vi "Variable glob alertes min-max temperatures.vi"() -> ()   [LabVIEW 2022 SP3]
panel:
  out "Groupe ON":bool[](array[boolean])
  out "Liste min/max temp":string[](array[string])
  in  "groupes min max temp":T1(array[cluster])
  in  "Al temp min/max en cours":bool
  # "Alertes min/max températures"
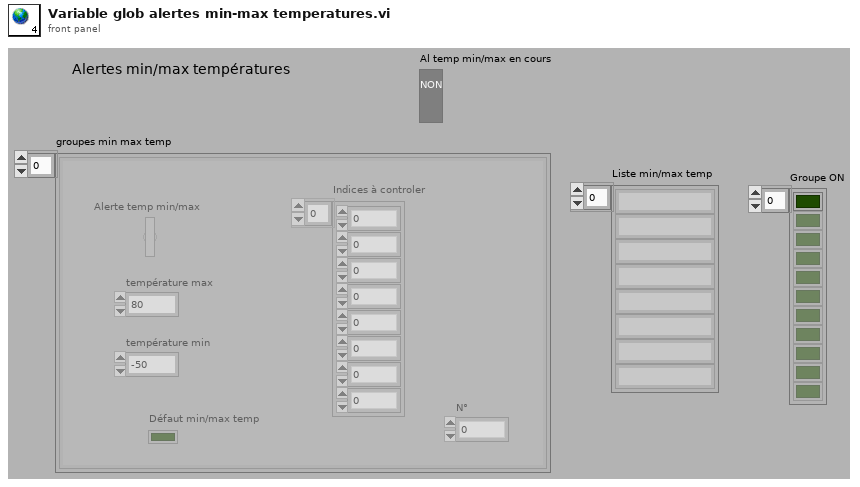
[diagram p1: front panel]
types:
  T1 = cluster{"Alerte temp min/max":bool, "température max":dbl, "température min":dbl, "Défaut min/max temp":bool, "Indices à controler":i16[], "N°":u16}[]
diagram:
